vi "load class.vi"(8 "error in":errorcluster, 9 "available class paths":path[](array[path]), 10 "available class names":string[](array[string]), 11 "Class Name":string) -> (0 "error out":errorcluster, 3 "Object Out":refnum<class>)   [LabVIEW 2014, in "class discovery singleton.lvlib"]
doc: "Attempts to load a class, by name, either from memory or from disk. First it tries the exact name in memory. Then it tries the filename on disk. Then it tries an approximate match of all VIs in memory."
uses:
  class discovery singleton.lvlib
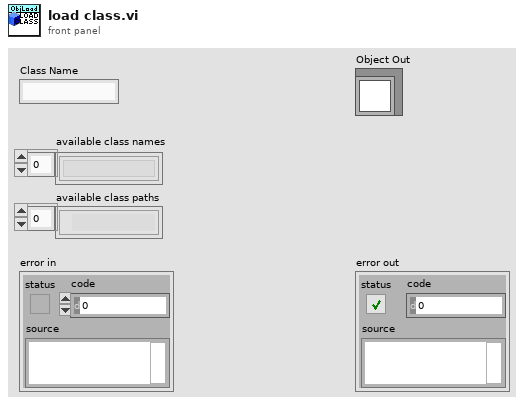
[diagram p1: front panel]
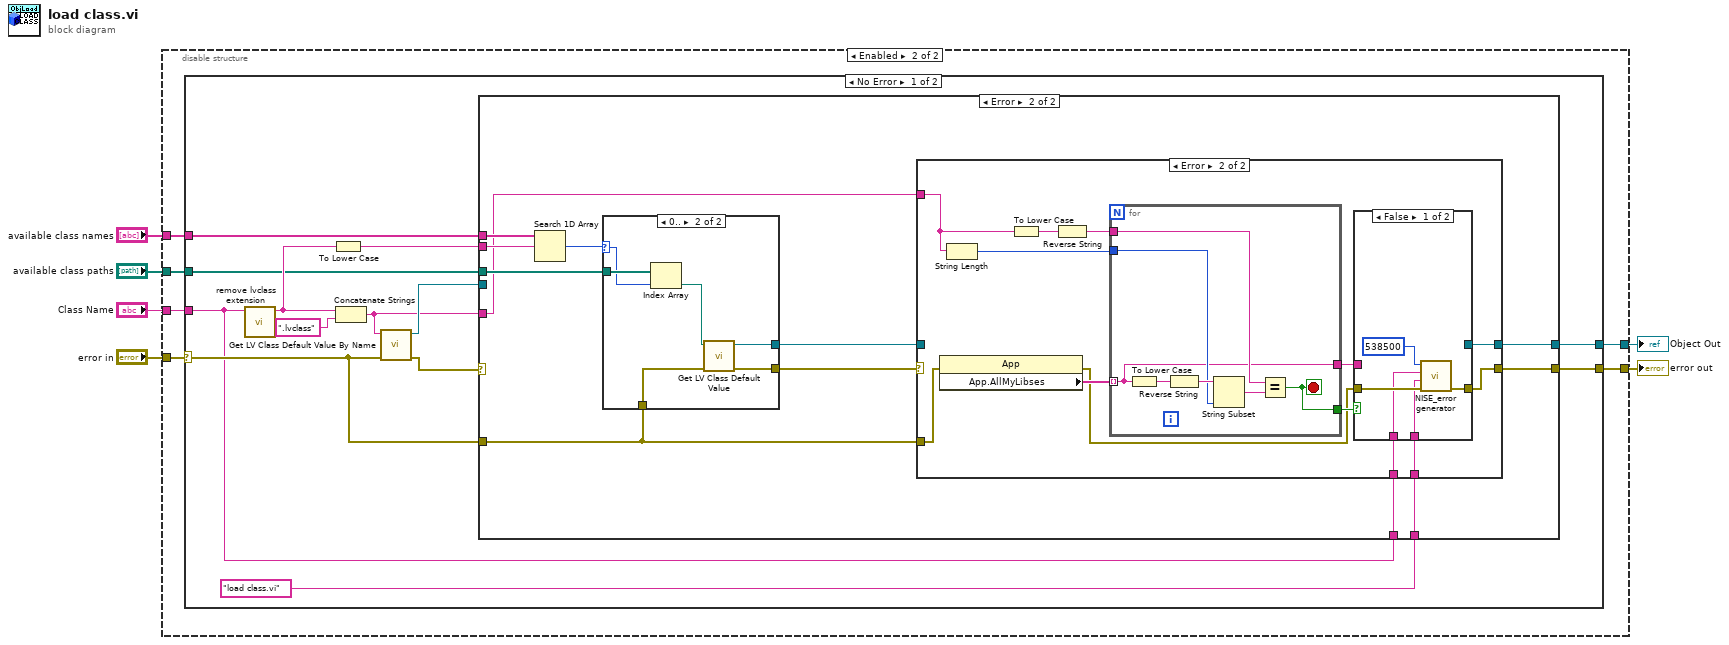
[diagram p0: block diagram]
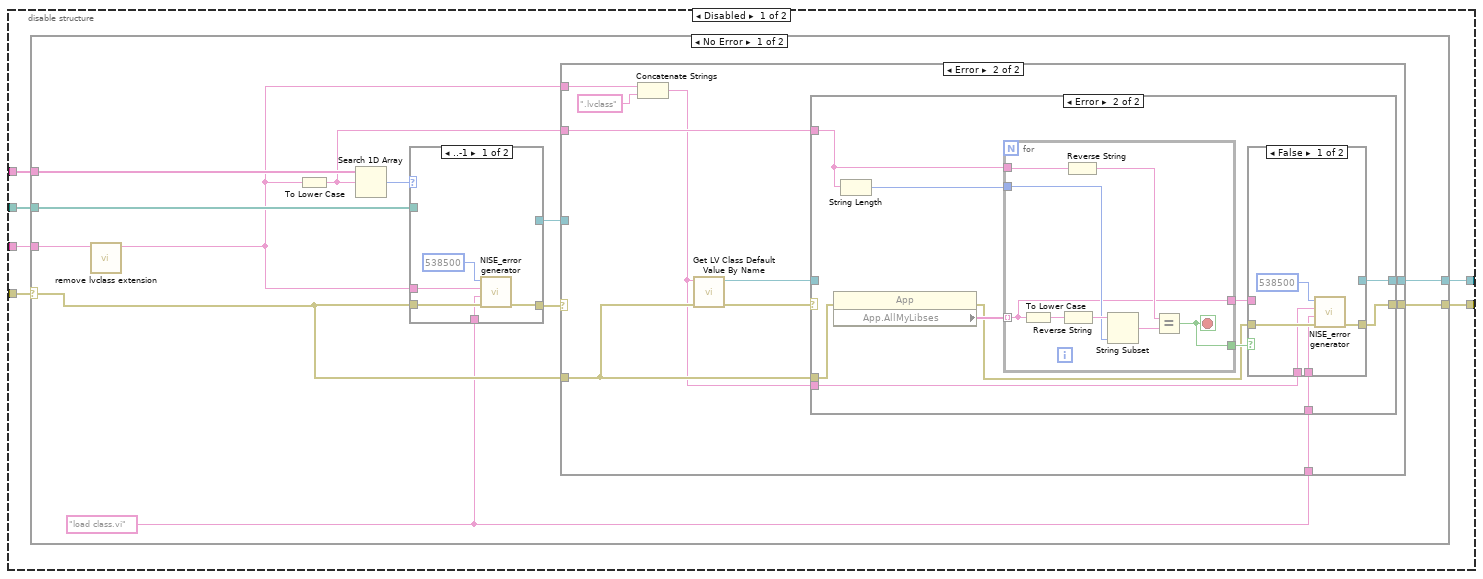
[diagram p2: hidden frame]
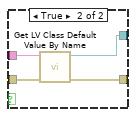
[diagram p5: hidden frame]
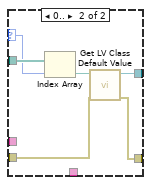
[diagram p6: hidden frame]
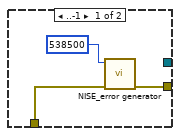
[diagram p9: hidden frame]
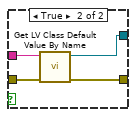
[diagram p11: hidden frame]
diagram:
  n1 = disable-structure shown="Enabled" {
    disable-tunnel: "Class Name" -> [w12 w84]
    disable-tunnel: "error in" -> [w11 w83]
    disable-tunnel: [w10 w82] -> w4
    disable-tunnel: [w9 w81] -> w3
    disable-tunnel: "available class paths" -> [w8 w80]
    disable-tunnel: "available class names" -> [w7 w79]
    frame Disabled {
      n2 = case shown="No Error" w11 {
        selector: w11 -> [w18 w78]
        tunnel: w12 -> [w22 _]
        tunnel: [w21 _] -> w9
        tunnel: [w19 w78] -> w10
        tunnel: w8 -> [w24 _]
        tunnel: w7 -> [w23 _]
        frame No Error {
          w13 = "load class.vi"
          n3 = call "remove lvclass extension.vi"("class name in"=w22) -> ("class name out"=w15:string)  [unwired: 10 in]
          n4 = To Lower Case(string=w15) -> (all lower case string=w14:string)
          n5 = Search 1D Array(1D array=w23, element=w14) -> (index of element=w17:i32)  [unwired: 1 in]
          n6 = case shown="..-1" w17 {
            selector: w17 -> [_ w73]
            tunnel: [w70 w77] -> w16
            tunnel: [_ w76] -> w20
            tunnel: w24 -> [_ w75]
            tunnel: w18 -> [w69 w72]
            tunnel: w15 -> [w68 _]
            tunnel: w13 -> [w67 _]
            frame ..-1 {
              n7 = call "NISE_error generator.vi"("error in"=w69, "source"=w67, "append error message"=w68, "error code (0)"=538500) -> ("error out"=w70:errorcluster)  [unwired: 5 in]
            }
            frame 0.. {
              n8 = Index Array(array=w75, index=w73) -> (element=w74:path)
              n9 = call <vilib>:"Get LV Class Default Value.vi"("error in (no error)"=w72, "class path"=w74) -> ("error out"=w77:errorcluster, "object"=w76:refnum<class>)  [unwired: 8 in]
            }
          }
          n10 = case shown="Error" w16 {
            selector: w16 -> [w25 _]
            tunnel: [w26 w36] -> w21
            tunnel: w20 -> [w26 _]
            tunnel: [w25 w35] -> w19
            tunnel: w15 -> [_ w33]
            tunnel: w18 -> [_ w34]
            tunnel: w14 -> [_ w29]
            tunnel: w13 -> [_ w27]
            frame No Error {
            }
            frame Error {
              n11 = Concatenate Strings(w33, ".lvclass" ("string")) -> (w28:string)
              n12 = call <vilib>:"Get LV Class Default Value By Name.vi"("error in (no error)"=w34, "class name"=w28) -> ("error out"=w31:errorcluster, "object"=w30:refnum<class>)  [unwired: 8 in]
              n13 = case shown="Error" w31 {
                selector: w31 -> [w38 _]
                tunnel: [w37 w42] -> w36
                tunnel: [w38 w43] -> w35
                tunnel: w34 -> [_ w49]
                tunnel: w28 -> [_ w41]
                tunnel: w30 -> [w37 _]
                tunnel: w29 -> [_ w40]
                tunnel: w27 -> [_ w39]
                frame No Error {
                }
                frame Error {
                  n14 = property class="App"(error in=w49) -> (error out=w44:errorcluster, "App.AllMyLibses"=w48:string[])  [unwired: 1 in, 1 out]
                  n15 = String Length(string=w40) -> (length=w47:i32)
                  n16 = for {
                    tunnel: w48 -> [w59] mode=indexing
                    tunnel: w40 -> [w66]
                    tunnel: w47 -> [w64]
                    tunnel: [w59] -> w46
                    tunnel: [w61] -> w45
                    stop <- w61 stop-if-true
                    n17 = To Lower Case(string=w59) -> (all lower case string=w60:string)
                    n18 = Reverse String(1:w60) -> (0:w65:string)
                    n19 = Reverse String(1:w66) -> (0:w62:string)
                    n20 = String Subset(string=w65, length (rest)=w64) -> (substring=w63:string)  [unwired: 1 in]
                    n21 = Equal?(x=w62, y=w63) -> (x = y?=w61:bool)
                  }
                  n22 = case shown="False" w45 {
                    tunnel: w46 -> [_ w58]
                    tunnel: w44 -> [w52 w57]
                    tunnel: [w53 w56] -> w43
                    tunnel: [_ w55] -> w42
                    tunnel: w41 -> [w51 _]
                    tunnel: w39 -> [w50 _]
                    frame False {
                      n23 = call "NISE_error generator.vi"("error in"=w52, "source"=w50, "append error message"=w51, "error code (0)"=538500) -> ("error out"=w53:errorcluster)  [unwired: 5 in]
                    }
                    frame True {
                      n24 = call <vilib>:"Get LV Class Default Value By Name.vi"("error in (no error)"=w57, "class name"=w58) -> ("error out"=w56:errorcluster, "object"=w55:refnum<class>)  [unwired: 8 in]
                    }
                  }
                }
              }
            }
          }
        }
        frame Error {
        }
      }
    }
    frame Enabled {
      n25 = case shown="No Error" w83 {
        selector: w83 -> [w93 w152]
        tunnel: w84 -> [w87 _]
        tunnel: [w97 _] -> w81
        tunnel: [w96 w152] -> w82
        tunnel: w80 -> [w86 _]
        tunnel: w79 -> [w88 _]
        frame No Error {
          n26 = call "remove lvclass extension.vi"("class name in"=w87) -> ("class name out"=w90:string)  [unwired: 10 in]
          n27 = To Lower Case(string=w90) -> (all lower case string=w95:string)
          n28 = Concatenate Strings(w90, ".lvclass" ("string")) -> (w85:string)
          n29 = call <vilib>:"Get LV Class Default Value By Name.vi"("error in (no error)"=w93, "class name"=w85) -> ("error out"=w92:errorcluster, "object"=w89:refnum<class>)  [unwired: 8 in]
          n30 = case shown="Error" w92 {
            selector: w92 -> [w98 _]
            tunnel: [w99 w111] -> w97
            tunnel: w89 -> [w99 _]
            tunnel: [w98 w110] -> w96
            tunnel: w93 -> [_ w109]
            tunnel: w95 -> [_ w104]
            tunnel: "load class.vi" -> [_ w106]
            tunnel: w88 -> [_ w105]
            tunnel: w87 -> [_ w103]
            tunnel: w86 -> [_ w101]
            tunnel: w85 -> [_ w100]
            frame No Error {
            }
            frame Error {
              n31 = Search 1D Array(1D array=w105, element=w104) -> (index of element=w102:i32)  [unwired: 1 in]
              n32 = case shown="0.." w102 {
                selector: w102 -> [_ w116]
                tunnel: w109 -> [w112 w120]
                tunnel: [w113 w119] -> w108
                tunnel: [_ w118] -> w107
                tunnel: w101 -> [_ w117]
                frame ..-1 {
                  n33 = call "NISE_error generator.vi"("error in"=w112, "error code (0)"=538500) -> ("error out"=w113:errorcluster)  [unwired: 7 in]
                }
                frame 0.. {
                  n34 = Index Array(array=w117, index=w116) -> (element=w115:path)
                  n35 = call <vilib>:"Get LV Class Default Value.vi"("error in (no error)"=w120, "class path"=w115) -> ("error out"=w119:errorcluster, "object"=w118:refnum<class>)  [unwired: 8 in]
                }
              }
              n36 = case shown="Error" w108 {
                selector: w108 -> [w122 _]
                tunnel: [w121 w128] -> w111
                tunnel: [w122 w129] -> w110
                tunnel: w109 -> [_ w135]
                tunnel: w107 -> [w121 _]
                tunnel: w100 -> [_ w127]
                tunnel: w106 -> [_ w126]
                tunnel: w103 -> [_ w125]
                frame No Error {
                }
                frame Error {
                  n37 = property class="App"(error in=w135) -> (error out=w130:errorcluster, "App.AllMyLibses"=w134:string[])  [unwired: 1 in, 1 out]
                  n38 = String Length(string=w127) -> (length=w133:i32)
                  n39 = To Lower Case(string=w127) -> (all lower case string=w124:string)
                  n40 = Reverse String(1:w124) -> (0:w123:string)
                  n41 = for {
                    tunnel: w134 -> [w145] mode=indexing
                    tunnel: w123 -> [w151]
                    tunnel: w133 -> [w149]
                    tunnel: [w145] -> w132
                    tunnel: [w147] -> w131
                    stop <- w147 stop-if-true
                    n42 = To Lower Case(string=w145) -> (all lower case string=w146:string)
                    n43 = Reverse String(1:w146) -> (0:w150:string)
                    n44 = String Subset(string=w150, length (rest)=w149) -> (substring=w148:string)  [unwired: 1 in]
                    n45 = Equal?(x=w151, y=w148) -> (x = y?=w147:bool)
                  }
                  n46 = case shown="False" w131 {
                    tunnel: w132 -> [_ w144]
                    tunnel: w130 -> [w138 w143]
                    tunnel: [w139 w142] -> w129
                    tunnel: [_ w141] -> w128
                    tunnel: w126 -> [w137 _]
                    tunnel: w125 -> [w136 _]
                    frame False {
                      n47 = call "NISE_error generator.vi"("error in"=w138, "source"=w137, "append error message"=w136, "error code (0)"=538500) -> ("error out"=w139:errorcluster)  [unwired: 5 in]
                    }
                    frame True {
                      n48 = call <vilib>:"Get LV Class Default Value By Name.vi"("error in (no error)"=w143, "class name"=w144) -> ("error out"=w142:errorcluster, "object"=w141:refnum<class>)  [unwired: 8 in]
                    }
                  }
                }
              }
            }
          }
        }
        frame Error {
        }
      }
    }
  }
  "error out" <- w4
  "Object Out" <- w3
